vi "DAC Init Results.vi"(8 "error in":errorcluster, 9 "Log Details?":bool, 10 "tdms file":refnum<k34>, 11 "DAC Traverse in":refnum<class "DAC Traverse.lvclass">) -> (0 "error out":errorcluster, 2 "tdms file out":refnum<k34>)   [LabVIEW 2019, in "DAC.lvlib" / "DAC Traverse.lvclass"]
uses:
  DAC Traverse.lvclass
  C:/Users/krio/Documents/LV_Projects/test-stand/App/DAC/DAC.lvclass
  DAC.lvclass/DAC.ctl
  DAC Traverse.lvclass/DAC Traverse.ctl
  DAC.lvclass
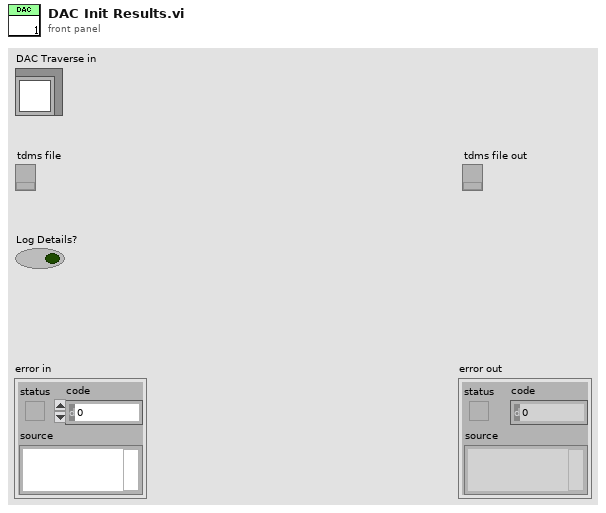
[diagram p1: front panel]
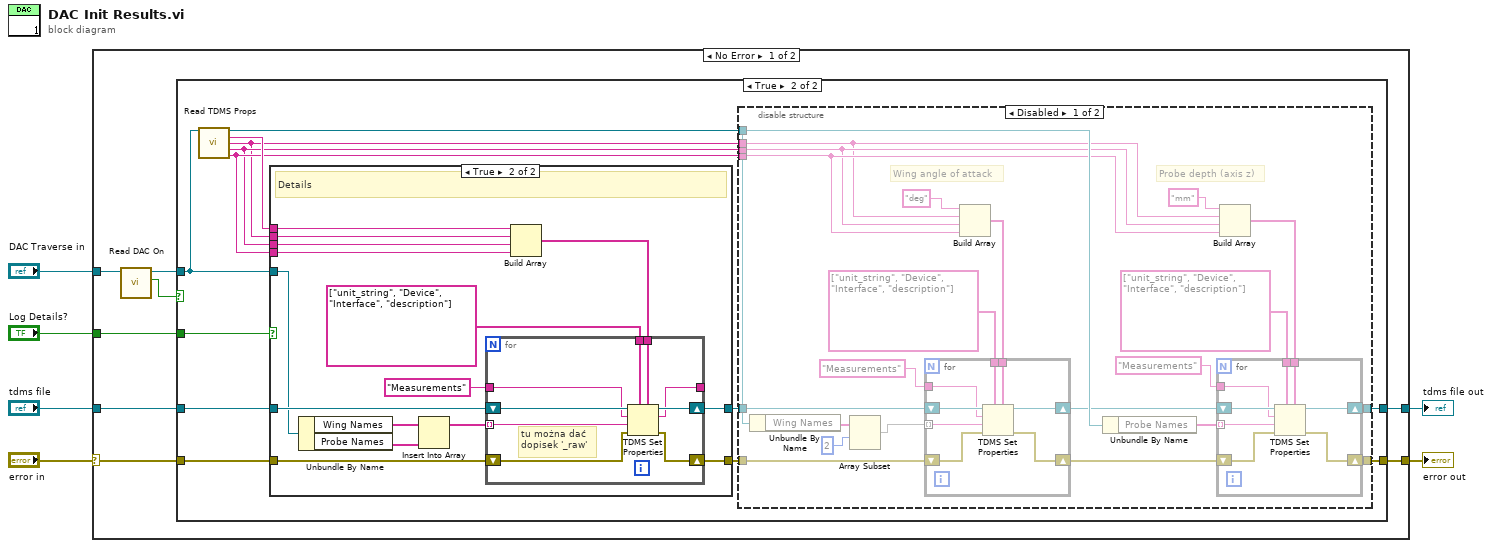
[diagram p0: block diagram]
diagram:
  n1 = case shown="No Error" "error in" {
    selector: "error in" -> [w8 w97]
    tunnel: [w12 w97] -> w3
    tunnel: "DAC Traverse in" -> [w11 _]
    tunnel: "tdms file" -> [w14 w96]
    tunnel: [w13 w96] -> w2
    tunnel: "Log Details?" -> [w7 _]
    frame No Error {
      n2 = call "Read DAC On.vi"("DAC in"=w11) -> ("DAC On"=w9:bool, "DAC out"=w10:refnum<class "DAC Traverse.lvclass">)  [unwired: 8 in, 1 out]
      n3 = case shown="True" w9 {
        tunnel: w14 -> [w16 w28]
        tunnel: [w16 w18] -> w13
        tunnel: [w15 w17] -> w12
        tunnel: w10 -> [_ w24]
        tunnel: w8 -> [w15 w25]
        tunnel: w7 -> [_ w29]
        frame False {
        }
        frame True {
          n4 = call "Read TDMS Props.vi"("DAC in"=w24) -> ("DAC out"=w23:refnum<class "DAC Traverse.lvclass">, "Result Unit"=w22:string, "DAC Device"=w19:string, "DAC IO"=w20:string, "DAC Description"=w21:string)  [unwired: 10 in]
          n5 = case shown="True" w29 {
            tunnel: w28 -> [w71 w86]
            tunnel: [w71 w75] -> w27
            tunnel: w24 -> [_ w85]
            tunnel: [w70 w74] -> w26
            tunnel: w25 -> [w70 w72]
            tunnel: w19 -> [_ w81]
            tunnel: w20 -> [_ w80]
            tunnel: w21 -> [_ w79]
            tunnel: w22 -> [_ w73]
            frame False {
            }
            frame True {
              # "Details"
              n6 = Unbundle By Name(w85) -> ("Wing Names"=w78:string[], "Probe Names"=w77:string[])
              n7 = Insert Into Array(array=w78, new element=w77) -> (w76:string[])  [unwired: 1 in]
              n8 = Build Array(w73, w81, w80, w79) -> (w82:string[])
              n9 = for {
                tunnel: string[] ["unit_string", "Device", "Interface", "description"] ("property names") -> [w94]
                tunnel: w82 -> [w93]
                shift-right: [w92] -> w75
                shift-left: w86 -> [w95]
                tunnel: "Measurements" ("group name in (Untitled)") -> [w90]
                shift-right: [w91] -> w74
                shift-left: w72 -> [w89]
                tunnel: w76 -> [w87] mode=indexing
                tunnel: [w88] -> _
                # "tu można dać\ndopisek '_raw'"
                n10 = TDMS Set Properties(5:w93, 7:w94, 8:w89, 9:w87, 10:w90, 11:w95) -> (0:w91:errorcluster, 2:w88:string, 3:w92:refnum<k34>)  [unwired: 1 out]
              }
            }
          }
          n11 = disable-structure shown="Disabled" {
            disable-tunnel: w27 -> [w51 w69]
            disable-tunnel: w26 -> [w49 w68]
            disable-tunnel: w23 -> [w41 _]
            disable-tunnel: w21 -> [w37 _]
            disable-tunnel: w20 -> [w36 _]
            disable-tunnel: w19 -> [w35 _]
            disable-tunnel: [w31 w69] -> w18
            disable-tunnel: [w30 w68] -> w17
            frame Disabled {
              # "Probe depth (axis z)"
              # "Wing angle of attack"
              n12 = Unbundle By Name(w41) -> ("Wing Names"=w46:string[])
              n13 = Array Subset(array=w46, index=2) -> (w40:string[])  [unwired: 1 in]
              n14 = Build Array("deg" ("element"), w35, w36, w37) -> (w47:string[])
              n15 = for {
                tunnel: w40 -> [w66] mode=indexing
                tunnel: string[] ["unit_string", "Device", "Interface", "description"] ("property names") -> [w65]
                tunnel: w47 -> [w64]
                shift-right: [w63] -> w33
                shift-left: w51 -> [w67]
                tunnel: "Measurements" ("group name in (Untitled)") -> [w61]
                shift-right: [w62] -> w32
                shift-left: w49 -> [w60]
                n16 = TDMS Set Properties(5:w64, 7:w65, 8:w60, 9:w66, 10:w61, 11:w67) -> (0:w62:errorcluster, 3:w63:refnum<k34>)  [unwired: 2 out]
              }
              n17 = Unbundle By Name(w41) -> ("Probe Names"=w38:string[])
              n18 = Build Array("mm" ("element"), w35, w36, w37) -> (w44:string[])
              n19 = for {
                tunnel: w38 -> [w58] mode=indexing
                tunnel: string[] ["unit_string", "Device", "Interface", "description"] ("property names") -> [w57]
                tunnel: w44 -> [w56]
                shift-right: [w55] -> w31
                shift-left: w33 -> [w59]
                tunnel: "Measurements" ("group name in (Untitled)") -> [w53]
                shift-right: [w54] -> w30
                shift-left: w32 -> [w52]
                n20 = TDMS Set Properties(5:w56, 7:w57, 8:w52, 9:w58, 10:w53, 11:w59) -> (0:w54:errorcluster, 3:w55:refnum<k34>)  [unwired: 2 out]
              }
            }
            frame Enabled {
            }
          }
        }
      }
    }
    frame Error {
    }
  }
  "error out" <- w3
  "tdms file out" <- w2
